vi "run state machine.vi"(8 "error in (no error)":errorcluster, 11 "SPARC4_GEI in":refnum<class "S4GEI.lvclass">) -> (0 "error out":errorcluster, 3 "SPARC4_GEI out":refnum<class "S4GEI.lvclass">)   [LabVIEW 2018, in "S4GEI.lvclass"]
uses:
  S4GEI.lvclass
  Channel GUI/Channel.lvclass
  State Machine/State Machine.lvclass
  TCS/TCS.lvclass
panel:
  in  "Header data":T1={"RA"="00:00:00", "DEC"="00:00:00", "EQUINOX"=0.0, "AIRMASS"=0.0, "TCSHA"="", "TCSDATE"="", "TELFOCUS"="", "EXTTEMP"="", "PRESSURE"="", "HUMIDITY"="", "ASEL"=FALSE, "CALW"="NONE", "WPSEL"="L2", "GFOC"=0, "GMIR"=0, "GUIDERA"="00:00:00", "GUIDEDEC"="00:00:00"}
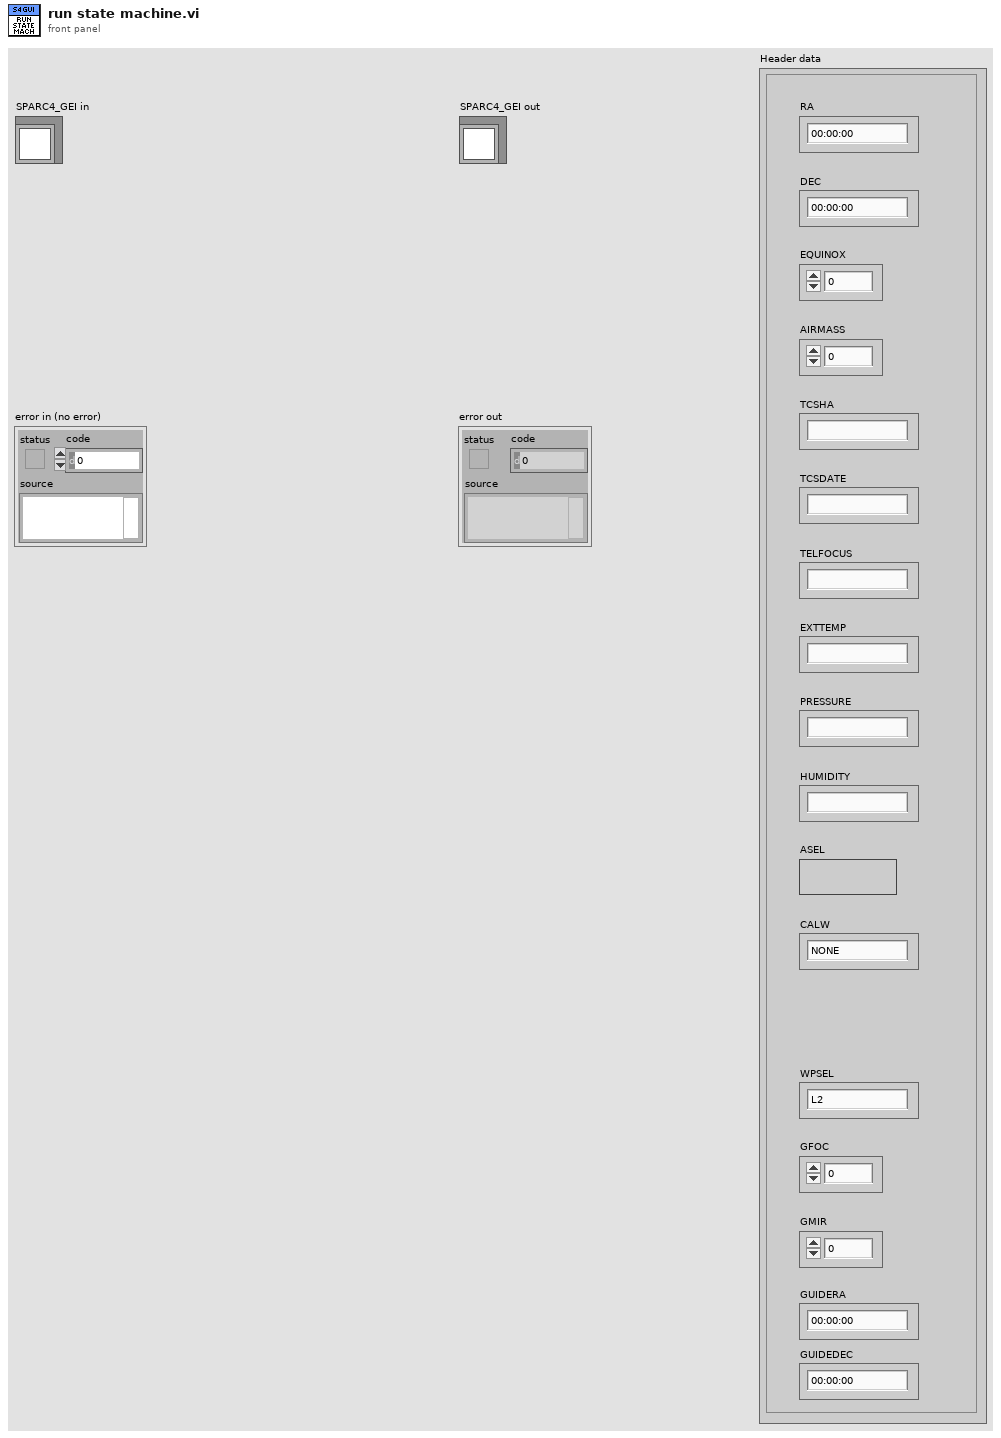
[diagram p1: front panel]
types:
  T1 = cluster{"RA":string, "DEC":string, "EQUINOX":dbl, "AIRMASS":dbl, "TCSHA":string, "TCSDATE":string, "TELFOCUS":string, "EXTTEMP":string, "PRESSURE":string, "HUMIDITY":string, "ASEL":bool, "CALW":string, "WPSEL":string, "GFOC":u16, "GMIR":u16, "GUIDERA":string, "GUIDEDEC":string}
  T2 = cluster{"OBJ":string, "RA":string, "DEC":string, "EQUINOX":dbl, "AIRMASS":dbl, "JD":dbl, "SD":string, "TCSHA":string, "TCSDATE":string, "TELFOCUS":string, "WS_DEFAULT":string, "EXTTEMP":string, "PRESSURE":string, "HUMIDITY":string}
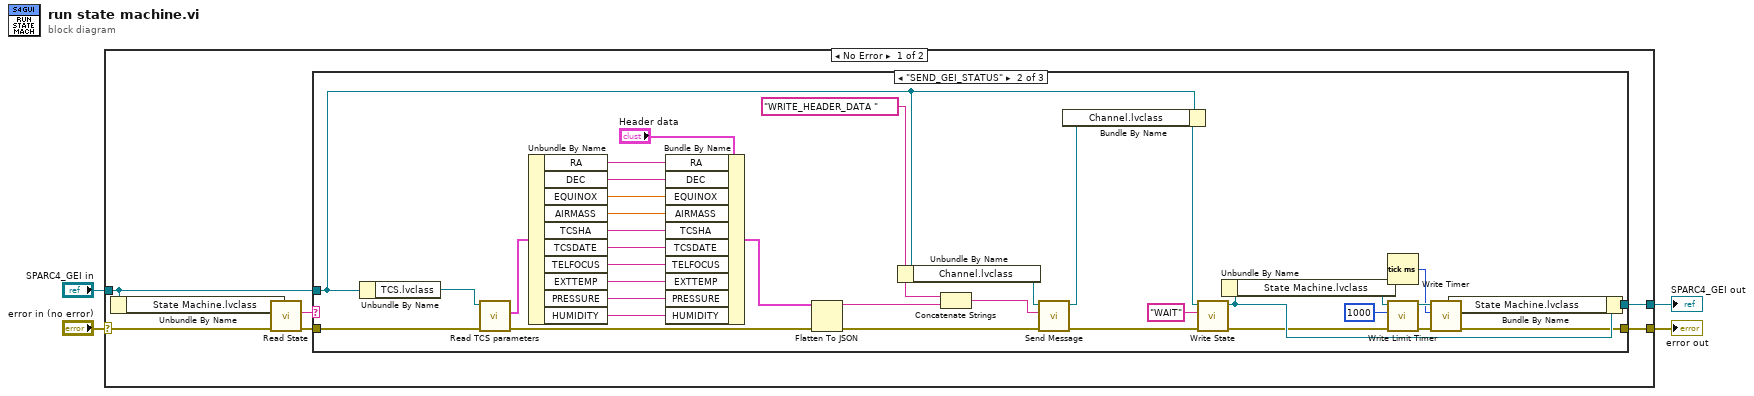
[diagram p0: block diagram]
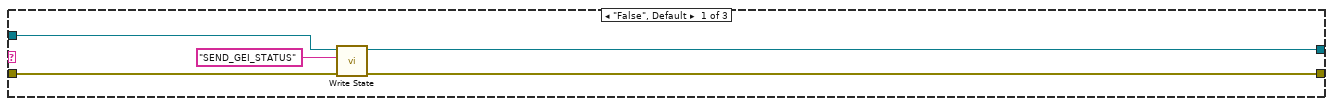
[diagram p2: hidden frame]
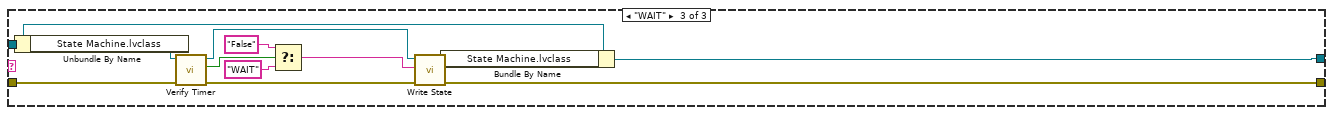
[diagram p3: hidden frame]
diagram:
  n1 = case shown="No Error" "error in (no error)" {
    selector: "error in (no error)" -> [w10 w66]
    tunnel: [w8 w66] -> w3
    tunnel: [w5 w65] -> w1
    tunnel: "SPARC4_GEI in" -> [w6 w65]
    frame No Error {
      n2 = Unbundle By Name(w6) -> ("State Machine.lvclass"=w11:refnum<class "State Machine.lvclass">)
      n3 = call-dynamic "Read State.vi"("error in (no error)"=w10, "State Machine in"=w11) -> ("error out"=w9:errorcluster, "State"=w7:string)  [unwired: 7 in, 1 out]
      n4 = case shown="\"SEND_GEI_STATUS\"" w7 {
        tunnel: w9 -> [w12 w50 w61]
        tunnel: [w14 w41 w59] -> w8
        tunnel: [w15 w44 w64] -> w5
        tunnel: w6 -> [w13 w49 w63]
        frame "False", Default {
          n5 = call "Write State.vi"("error in (no error)"=w12, "State"="SEND_GEI_STATUS", "SPARC4_GEI in"=w13) -> ("error out"=w14:errorcluster, "SPARC4_GEI out"=w15:refnum<class "S4GEI.lvclass">)  [unwired: 7 in]
        }
        frame "SEND_GEI_STATUS" {
          n6 = Unbundle By Name(w49) -> ("TCS.lvclass"=w33:refnum<class "TCS.lvclass">)
          n7 = call-dynamic "Read TCS parameters.vi"("error in (no error)"=w50, "TCS in"=w33) -> ("error out"=w19:errorcluster, "TCS parameters"=w31:T2)  [unwired: 7 in, 1 out]
          n8 = Unbundle By Name(w31) -> ("RA"=w21:string, "DEC"=w22:string, "EQUINOX"=w23:dbl, "AIRMASS"=w24:dbl, "TCSHA"=w25:string, "TCSDATE"=w26:string, "TELFOCUS"=w27:string, "EXTTEMP"=w28:string, "PRESSURE"=w29:string, "HUMIDITY"=w30:string)
          n9 = Bundle By Name(cluster="Header data", "RA"=w21, "DEC"=w22, "EQUINOX"=w23, "AIRMASS"=w24, "TCSHA"=w25, "TCSDATE"=w26, "TELFOCUS"=w27, "EXTTEMP"=w28, "PRESSURE"=w29, "HUMIDITY"=w30) -> (w20:T1)
          n10 = Flatten To JSON(anything=w20, error in (no error)=w19) -> (JSON string=w17:string, 11:w18:errorcluster)  [unwired: 1 in]
          n11 = Unbundle By Name(w49) -> ("Channel.lvclass"=w52:refnum<class "Channel.lvclass">)
          n12 = Concatenate Strings("WRITE_HEADER_DATA ", w17) -> (w35:string)
          n13 = call "Send Message.vi"("error in (no error)"=w18, "Message"=w35, "Channel GUI in"=w52) -> ("error out"=w47:errorcluster, "Channel GUI out"=w51:refnum<class "Channel.lvclass">)  [unwired: 7 in]
          n14 = Bundle By Name(cluster=w49, "Channel.lvclass"=w51) -> (w48:refnum<class "S4GEI.lvclass">)
          n15 = call "Write State.vi"("error in (no error)"=w47, "State"="WAIT", "SPARC4_GEI in"=w48) -> ("error out"=w39:errorcluster, "SPARC4_GEI out"=w45:refnum<class "S4GEI.lvclass">)  [unwired: 7 in]
          n16 = Unbundle By Name(w45) -> ("State Machine.lvclass"=w38:refnum<class "State Machine.lvclass">)
          n17 = Tick Count (ms)() -> (millisecond timer value=w36:u32)
          n18 = call "Write Limit Timer.vi"("error in (no error)"=w39, "Limit Timer"=u32 1000, "State Machine in"=w38) -> ("error out"=w40:errorcluster, "State Machine out"=w43:refnum<class "State Machine.lvclass">)  [unwired: 7 in]
          n19 = call "Write Timer.vi"("error in (no error)"=w40, "Timer"=w36, "State Machine in"=w43) -> ("error out"=w41:errorcluster, "State Machine out"=w42:refnum<class "State Machine.lvclass">)  [unwired: 7 in]
          n20 = Bundle By Name(cluster=w45, "State Machine.lvclass"=w42) -> (w44:refnum<class "S4GEI.lvclass">)
        }
        frame "WAIT" {
          n21 = Unbundle By Name(w63) -> ("State Machine.lvclass"=w62:refnum<class "State Machine.lvclass">)
          n22 = call "Verify Timer.vi"("error in (no error)"=w61, "State Machine in"=w62) -> ("error out"=w55:errorcluster, "time out"=w58:bool, "State Machine out"=w56:refnum<class "State Machine.lvclass">)  [unwired: 7 in]
          n23 = Select(t="False", s=w58, f="WAIT") -> (s? t:f=w57:string)
          n24 = call-dynamic "Write State.vi"("error in (no error)"=w55, "State"=w57, "State Machine in"=w56) -> ("error out"=w59:errorcluster, "State Machine out"=w60:refnum<class "State Machine.lvclass">)  [unwired: 7 in]
          n25 = Bundle By Name(cluster=w63, "State Machine.lvclass"=w60) -> (w64:refnum<class "S4GEI.lvclass">)
        }
      }
    }
    frame Error {
    }
  }
  "error out" <- w3
  "SPARC4_GEI out" <- w1
